vi "Own20261012_SetConnectorPattern.vi"() -> ()   [LabVIEW 2024]
panel:
  in  "pattern":u32
  out "error out":errorcluster caption="错误输出"
  in  "target_path":path
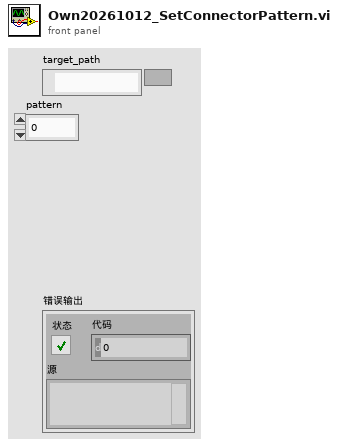
[diagram p1: front panel]
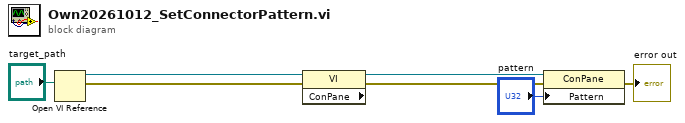
[diagram p0: block diagram]
diagram:
  n1 = Open VI Reference ("打开VI引用")(vi path="target_path") -> (vi reference=w6:refnum<vi>, error out=w5:errorcluster)  [unwired: 5 in]
  n2 = property on="属性节点" class="VI"(reference=w6, error in=w5) -> (error out=w3:errorcluster, "ConPane"=w4:refnum<vi>)  [unwired: 1 out]
  n3 = property on="属性节点" class="ConPane"(reference=w4, error in=w3, "Pattern"="pattern") -> (error out=→"error out":errorcluster)  [unwired: 1 out]
